vi "WriteAO.vi"(8 "error in (no error)":errorcluster, 9 "PWM Settings":T1, 10 "Analog Output":T2, 11 "VISA resource name":refnum<visa-resource-name>) -> (0 "error out":errorcluster, 3 "VISA resource name out":refnum<visa-resource-name>)   [LabVIEW 2020, in "HandsOnPi2040.lvlib"]
doc: "Establishes communication with the instrument and optionally performs an instrument identification query and/or an instrument reset. It also places the instrument in a default state needed for other instrument driver operations. Therefore, call this VI before calling other instrument driver VIs for this instrument. Generally, you need to call the <b>Initialize</b> VI only once at the beginning of an application."
uses:
  HandsOnPi2040.lvlib
  cti-drivers-lv-visa-main/CTI-Visa/CTI-Visa.lvlib
  AOs.ctl
  PWMSettings.ctl
panel:
  # "Output"
  # "Input"
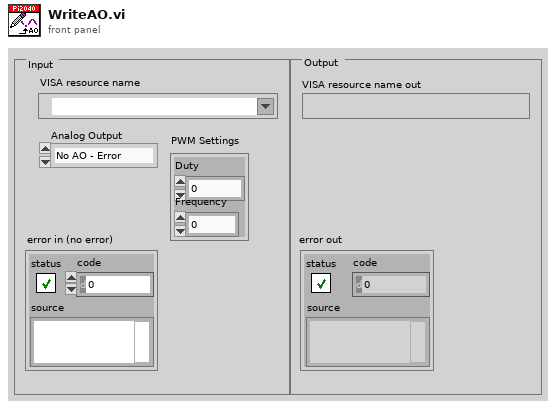
[diagram p1: front panel]
types:
  T1 = typedef "HandsOnPi2040.lvlib/PWMSettings.ctl" = cluster{"Duty":sgl, "Frequency":sgl}
  T2 = typedef "HandsOnPi2040.lvlib/AOs.ctl" = enum16{"No AO - Error", "AO1 (GPIO28)"}
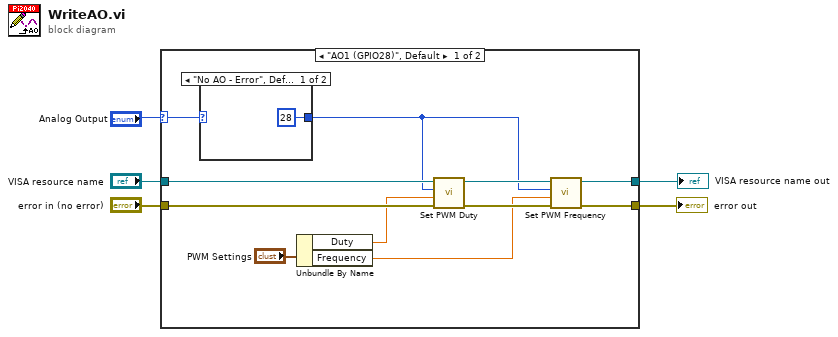
[diagram p0: block diagram]
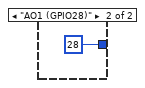
[diagram p2: hidden frame]
diagram:
  n1 = case shown="\"AO1 (GPIO28)\", Default" "Analog Output" {
    selector: "Analog Output" -> [w10 _]
    tunnel: [w13 w20] -> w4
    tunnel: [w14 w19] -> w5
    tunnel: "VISA resource name" -> [w16 w19]
    tunnel: "error in (no error)" -> [w12 w20]
    frame "AO1 (GPIO28)", Default {
      n2 = case shown="\"No AO - Error\", Default" w10 {
        tunnel: [28 ("Channel") 28 ("Channel")] -> w9
        frame "No AO - Error", Default {
        }
        frame "AO1 (GPIO28)" {
        }
      }
      n3 = Unbundle By Name("PWM Settings") -> ("Duty"=w7:sgl, "Frequency"=w6:sgl)
      n4 = call "Set PWM Duty.vi"("error in (no error)"=w12, "Duty % (0-1)"=w7, "Channel"=w9, "VISA resource name in"=w16) -> ("error out"=w11:errorcluster, "VISA resource name"=w15:refnum<visa-resource-name>)  [unwired: 6 in]
      n5 = call "Set PWM Frequency.vi"("error in (no error)"=w11, "Freq Hz"=w6, "Channel"=w9, "VISA resource name in"=w15) -> ("error out"=w13:errorcluster, "VISA resource name"=w14:refnum<visa-resource-name>)  [unwired: 6 in]
    }
    frame "No AO - Error" {
    }
  }
  "VISA resource name out" <- w5
  "error out" <- w4
